vi "Module Loop.vi"(8 "error in (no error)":errorcluster, 11 "DAQmxDI in":refnum<class "DAQmxDI.lvclass">) -> (0 "error out":errorcluster, 3 "DAQmxDI out":refnum<class "DAQmxDI.lvclass">)   [LabVIEW 2020, in "VolatusDAQ.lvlib" / "DAQmxDI.lvclass"]
uses:
  DAQmxDI.lvclass
  C:/dev/lv20CE/relink/lv-volatus/Volatus/Module/Module.lvclass
  Volatus/Module/Module.lvclass/Module.ctl
  Volatus/MessageQ/MessageQ.lvclass/MessageQ.ctl
  DAQmxDI.lvclass/DAQmxDI.ctl
  Volatus/Module/Module.lvclass
  <vilib>/Utility/error.llb/Error Cluster From Error Code.vi
  Volatus/MessageQ/MessageQ.lvclass
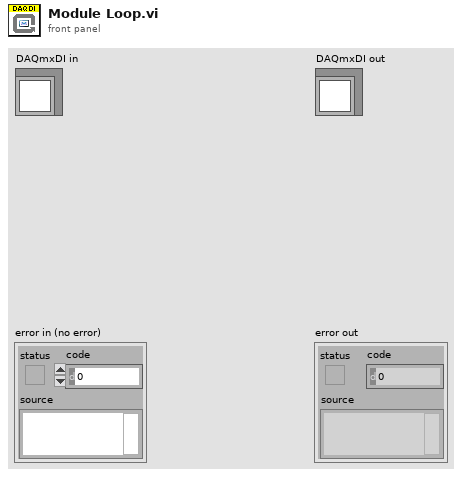
[diagram p1: front panel]
types:
  T1 = enum32{"Invalid", "Standard", "Closed", "Hidden", "Minimized", "Maximized"}
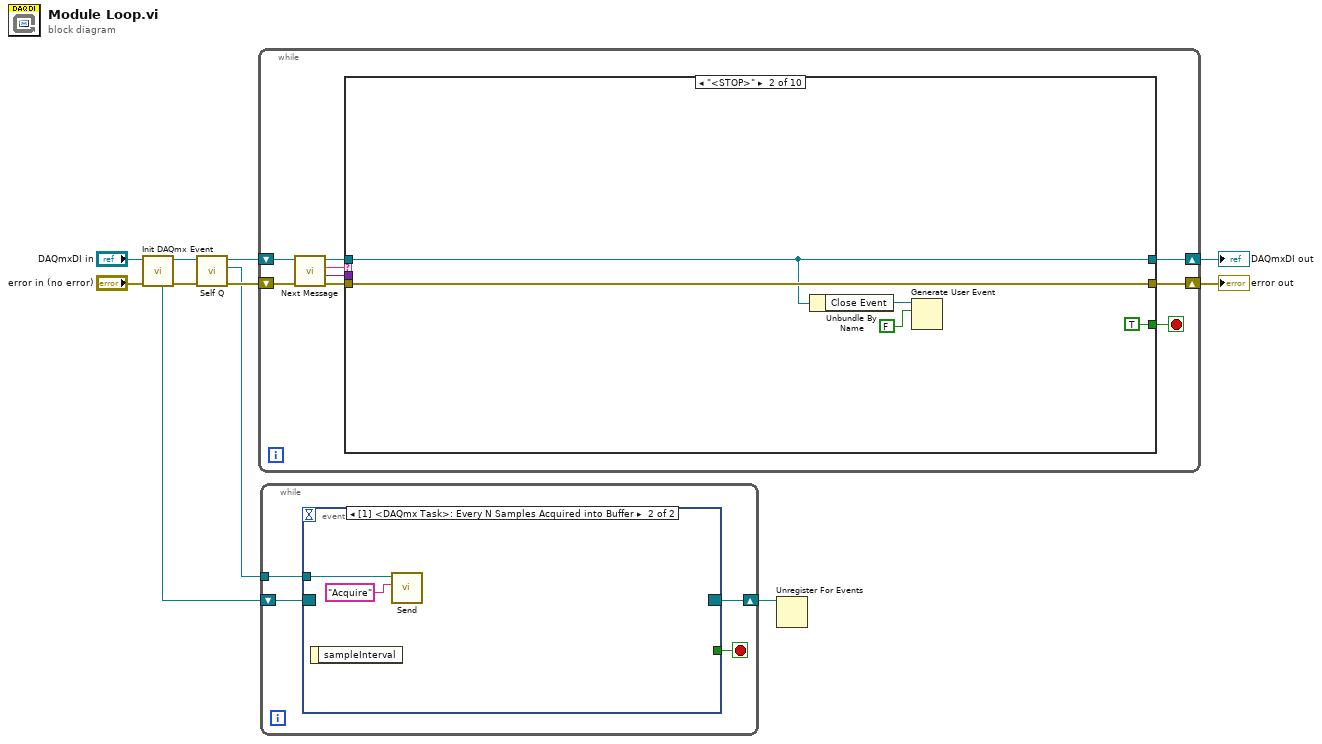
[diagram p0: block diagram]
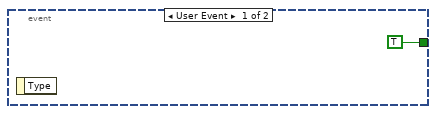
[diagram p2: hidden frame]
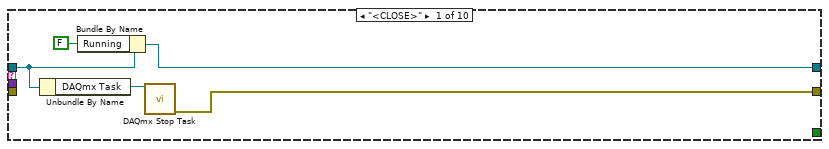
[diagram p3: hidden frame]
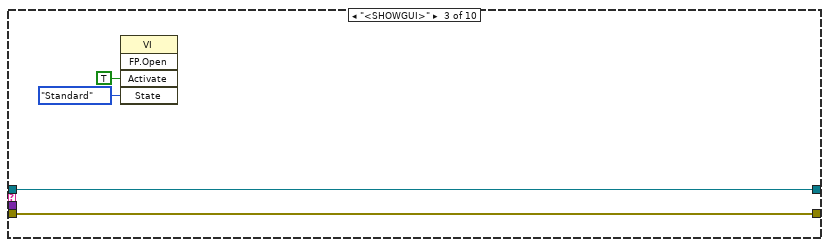
[diagram p4: hidden frame]
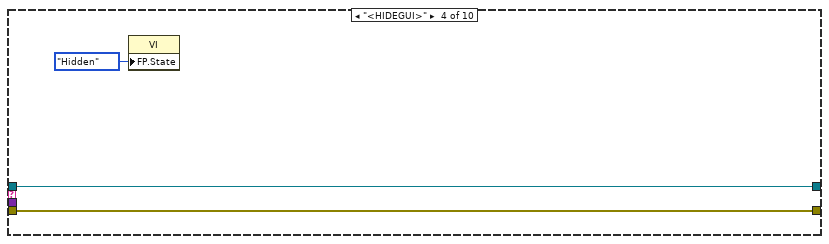
[diagram p5: hidden frame]
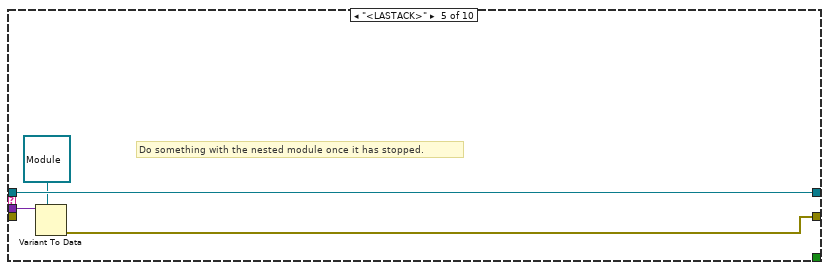
[diagram p6: hidden frame]
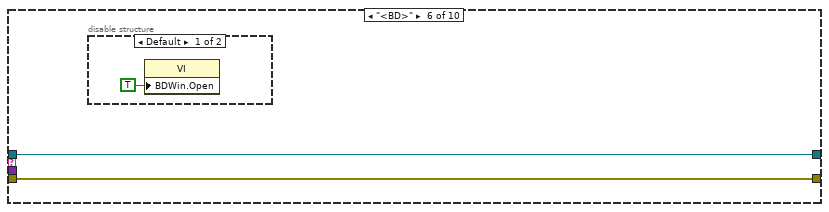
[diagram p7: hidden frame]
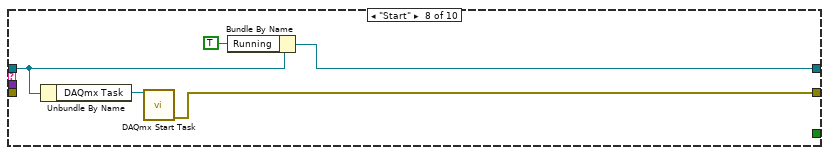
[diagram p10: hidden frame]
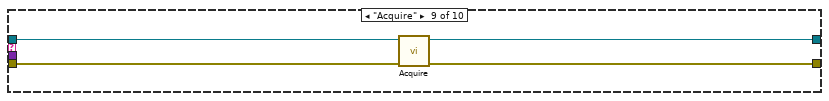
[diagram p11: hidden frame]
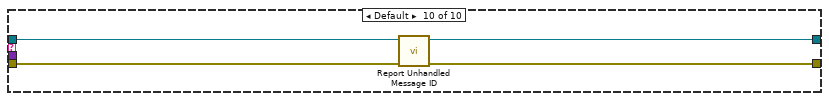
[diagram p12: hidden frame]
diagram:
  n1 = call "Init DAQmx Event.vi"("error in (no error)"="error in (no error)", "DAQmxDI in"="DAQmxDI in") -> ("error out"=w6:errorcluster, "DAQmxDI out"=w4:refnum<class "DAQmxDI.lvclass">, "Event Reg"=w3:refnum<event-registration>)  [unwired: 7 in]
  n2 = call "Self Q.vi"("Module in"=w4) -> ("Self Q"=w1:refnum<class "MessageQ.lvclass">, "Module out"=w2:refnum<class "DAQmxDI.lvclass">)  [unwired: 9 in]
  n3 = while {
    shift-right: [w14] -> w9
    shift-left: w2 -> [w19]
    shift-right: [w13] -> w8
    shift-left: w6 -> [w18]
    stop <- w12 stop-if-true
    n4 = call "Next Message.vi"("error in (no error)"=w18, "Module in"=w19) -> ("error out"=w17:errorcluster, "Data"=w11:variant, "ID"=w16:string, "Module out"=w15:refnum<class "DAQmxDI.lvclass">)  [unwired: 6 in]
    n5 = case shown="\"<STOP>\"" w16 {
      tunnel: w17 -> [_ w29 w32 w35 _ w41 w45 _ w54 w58]
      tunnel: w15 -> [w23 w27 w33 w36 w40 w42 w44 w50 w52 w56]
      tunnel: [w21 w27 w33 w36 w40 w42 w44 w47 w51 w55] -> w14
      tunnel: [w22 w29 w32 w35 w37 w41 w45 w48 w53 w57] -> w13
      tunnel: [_ TRUE _ _ _ _ _ _ _ _] -> w12
      tunnel: w11 -> [_ _ _ _ w39 _ _ _ _ _]
      frame "<CLOSE>" {
        n6 = Unbundle By Name(w23) -> ("DAQmx Task"=w24:refnum<k21>)
        n7 = Bundle By Name(cluster=w23, "Running"=FALSE) -> (w21:refnum<class "DAQmxDI.lvclass">)
        n8 = call <vilib>:"DAQmx Stop Task.vi"("task/channels in"=w24) -> ("error out"=w22:errorcluster)  [unwired: 13 in, 1 out]
      }
      frame "<STOP>" {
        n9 = Unbundle By Name(w27) -> ("Close Event"=w26:refnum<user-event>)
        n10 = Generate User Event(user event=w26, event data cluster=FALSE ("event data")) -> ()  [unwired: 2 in, 2 out]
      }
      frame "<SHOWGUI>" {
        n11 = invoke class="VI" method="FP.Open"("Activate"=TRUE ("Activate?"), "State"=T1."Standard") -> ()  [unwired: 3 in, 5 out]
      }
      frame "<HIDEGUI>" {
        n12 = property class="VI"("FP.State"=T1."Hidden" ("Front Panel Window:State")) -> ()  [unwired: 2 in, 2 out]
      }
      frame "<LASTACK>" {
        # "Do something with the nested module once it has stopped."
        n13 = Variant To Data(type=refnum<class "Module.lvclass"> refnum ("Volatus:Module"), Variant=w39) -> (error out=w37:errorcluster)  [unwired: 1 in, 1 out]
      }
      frame "<BD>" {
        n14 = disable-structure shown="Default" {
          frame condition #0 (active) {
            n15 = property class="VI"("BDWin.Open"=TRUE ("Block Diagram Window:Open")) -> ()  [unwired: 2 in, 2 out]
          }
          frame condition #1 {
          }
        }
      }
      frame "<TIMEOUT>" {
        # "No message for this module was received in time"
      }
      frame "Start" {
        n16 = Unbundle By Name(w50) -> ("DAQmx Task"=w49:refnum<k21>)
        n17 = call <vilib>:"DAQmx Start Task.vi"("task/channels in"=w49) -> ("error out"=w48:errorcluster)  [unwired: 13 in, 1 out]
        n18 = Bundle By Name(cluster=w50, "Running"=TRUE) -> (w47:refnum<class "DAQmxDI.lvclass">)
      }
      frame "Acquire" {
        n19 = call "Acquire.vi"("error in (no error)"=w54, "DAQmxDI in"=w52) -> ("error out"=w53:errorcluster, "DAQmxDI out"=w51:refnum<class "DAQmxDI.lvclass">)  [unwired: 8 in]
      }
      frame Default {
        n20 = call "Report Unhandled Message ID.vi"("error in (no error)"=w58, "Module in"=w56) -> ("error out"=w57:errorcluster, "Module out"=w55:refnum<class "DAQmxDI.lvclass">)  [unwired: 8 in]
      }
    }
  }
  "error out" <- w8
  "DAQmxDI out" <- w9
  n21 = while {
    tunnel: w1 -> [w61]
    shift-right: [w60] -> w7
    shift-left: w3 -> [w62]
    stop <- w59 stop-if-true
    n22 = event shown="[1] <DAQmx Task>: Every N Samples Acquired into Buffer" {
      selector: w62 -> [_ _]
      dyn-events: [_ _] -> w60
      timeout: _ -> [_ _]
      tunnel: w61 -> [_ w65]
      tunnel: [TRUE _] -> w59
      event User Event {
        n23 = event-data() -> ()  [unwired: 1 in, 1 out]
      }
      event Every N Samples Acquired into Buffer {
        n24 = event-data() -> ()  [unwired: 1 in, 1 out]
        n25 = call "Send.vi"("ID"="Acquire", "MessageQ in"=w65) -> ()  [unwired: 8 in, 2 out]
      }
    }
  }
  n26 = Unregister For Events(event registration refnum=w7) -> ()  [unwired: 1 in, 1 out]
